vi "Configuration Files.vi"(8 "error in (no error)":errorcluster, 11 "Node Ptr":T3 format="%.0x") -> (0 "error out":errorcluster)   [LabVIEW 2020, in "Ballard ARINC 429 System Explorer.lvlib" / "Implementation.lvlib"]
uses:
  Implementation.lvlib
  <vilib>/NI VeriStand/Custom Device API/Custom Device API.lvlib
  <vilib>/NI VeriStand/Custom Device Tools/Custom Device Utility Library/Custom Device Utility Library.lvlib
  Types/Browse Button.ctl
  Types/Path Control.ctl
  Scripting/Ballard/Ballard ARINC 429 Scripting.lvlib
  <vilib>/NI VeriStand/Custom Device API/Custom Device Item Ref.ctl
  Types/Configuration Files Page Data.ctl
panel:
  in  "Refresh":bool
  in  "Parameters":T1
  in  "Hardware":T1
  in  "SHDocVw.IWebBrowser":refnum<k7>(container)
  in  "General Header":cluster{"Section Name":string}={"Section Name"="Ballard ARINC 429 - Configuration Files"}
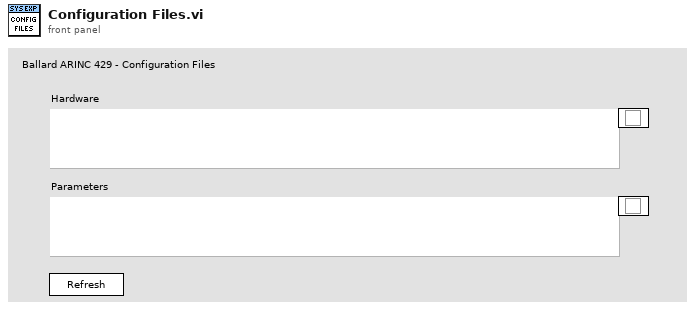
[diagram p1: front panel]
types:
  T1 = typedef "Ballard ARINC 429 System Explorer.lvlib/Implementation.lvlib/Path Control.ctl" = cluster{"file path":path, "Browse":T2}
  T2 = typedef "Ballard ARINC 429 System Explorer.lvlib/Implementation.lvlib/Browse Button.ctl" = bool
  T3 = typedef "Custom Device API.lvlib/Custom Device Item Ref.ctl" = u64
  T4 = typedef "Ballard ARINC 429 System Explorer.lvlib/Implementation.lvlib/Configuration Files Page Data.ctl" = cluster{"Hardware":T1, "Parameters":T1, "most recent parameters path":path, "most recent hardware path":path, "custom device ref":T3, "MD5":string, "CD scripted?":bool, "parameters path ctl ref":refnum<vi>}
  T5 = typedef "Custom Device API.lvlib/Custom Device Commands.ctl" = enum16{"Default", "Item renamed", "Shutdown", "Dynamic button pressed"}
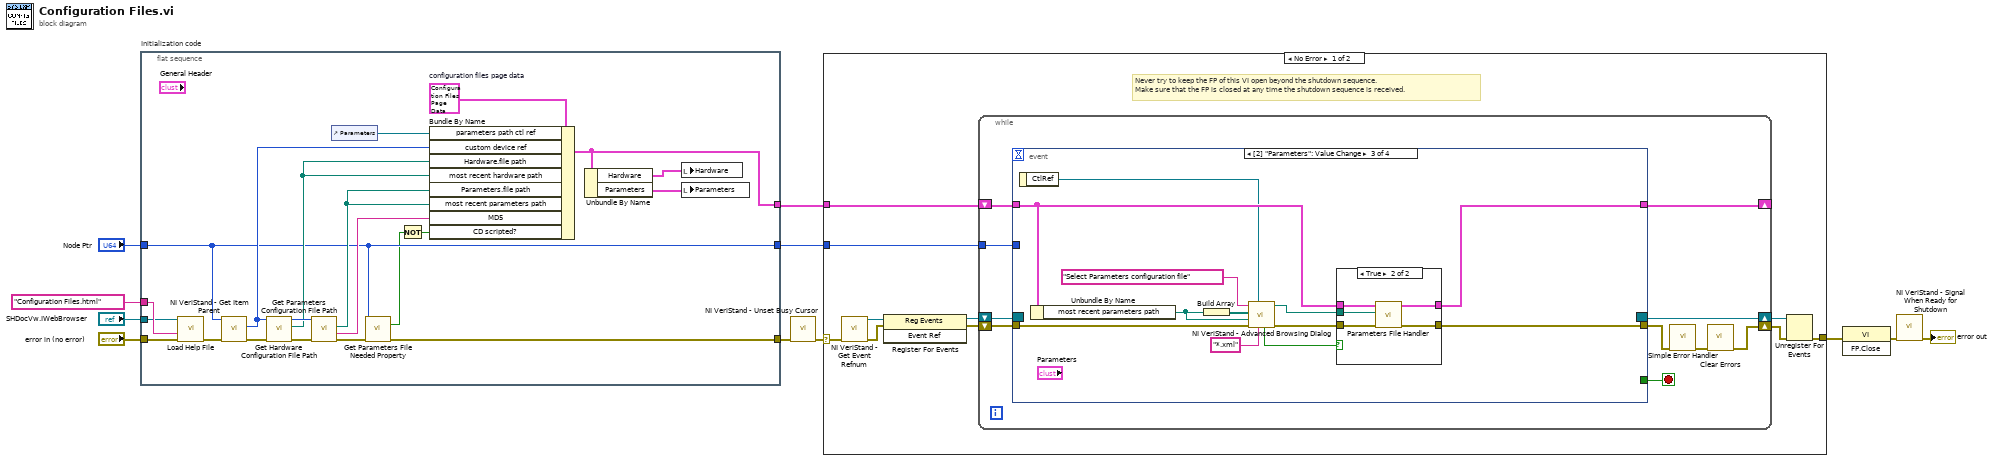
[diagram p0: block diagram]
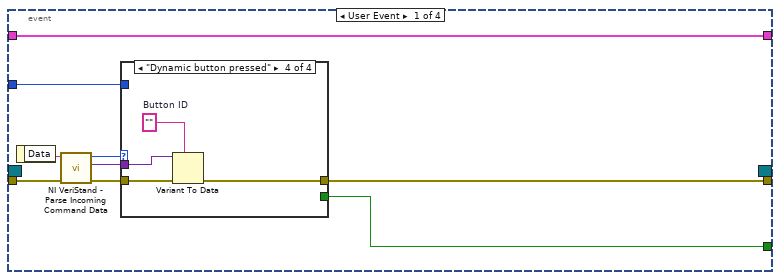
[diagram p2: hidden frame]
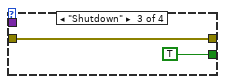
[diagram p5: hidden frame]
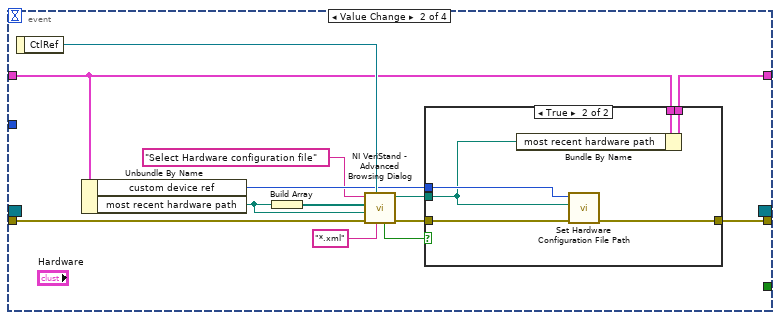
[diagram p6: hidden frame]
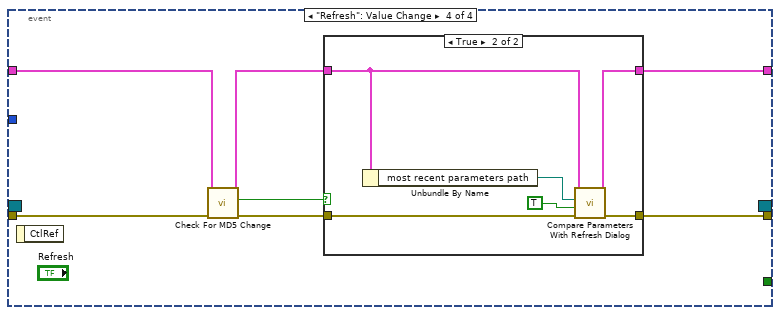
[diagram p9: hidden frame]
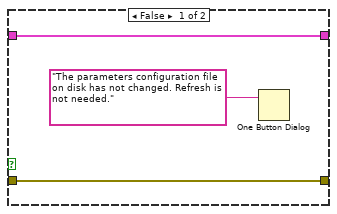
[diagram p10: hidden frame]
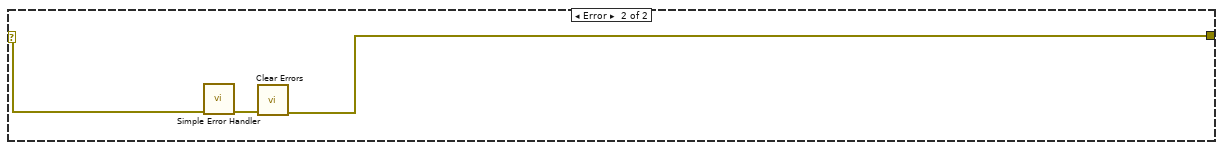
[diagram p11: hidden frame]
diagram:
  n1 = flat-sequence "Initialization code" {
    tunnel: "error in (no error)" -> [w32]
    tunnel: "Node Ptr" -> [w14]
    tunnel: [w15] -> w7
    tunnel: [w14] -> w4
    tunnel: "SHDocVw.IWebBrowser" -> [w21]
    tunnel: "Configuration Files.html" ("CD_CHM_Section") -> [w31]
    tunnel: [w19] -> w1
    frame #0 {
      w30 = T4 {"Hardware"={"file path"=path "", "Browse"=FALSE}, "Parameters"={"file path"=path "", "Browse"=FALSE}, "most recent parameters path"=path "", "most recent hardware path"=path "", "custom device ref"=0, "MD5"="", "CD scripted?"=FALSE, "parameters path ctl ref"=refnum}  # configuration files page data
      n2 = call "Load Help File.vi"("error in (no error)"=w32, "HTML File to Load"=w31, "Browser"=w21) -> ("error out"=w24:errorcluster)  [unwired: 8 in]
      n3 = call <vilib>:"NI VeriStand - Get Item Parent.vi"("error in (no error)"=w24, "Item Ref in"=w14) -> ("error out"=w23:errorcluster, "Parent Ref"=w22:T3)  [unwired: 6 in, 2 out]
      n4 = call "Get Hardware Configuration File Path.vi"("error in"=w23, "Ballard ARINC 429 custom device in"=w22) -> ("error out"=w26:errorcluster, "hardware configuration file path"=w25:path, "Ballard ARINC 429 custom device out"=w27:T3)  [unwired: 6 in, 1 out]
      n5 = call "Get Parameters Configuration File Path.vi"("error in"=w26, "Ballard ARINC 429 custom device in"=w27) -> ("error out"=w16:errorcluster, "MD5 checksum"=w18:string, "parameters configuration file path"=w20:path)  [unwired: 6 in, 1 out]
      n6 = control-ref of="Parameters"() -> (w17:refnum<vi>)
      n7 = call "Get Parameters File Needed Property.vi"("error in"=w16, "configuration files ref"=w14) -> ("error out"=w15:errorcluster, "needed"=w13:bool)  [unwired: 7 in, 1 out]
      n8 = Not(x=w13) -> (.not. x?=w12:bool)
      n9 = Bundle By Name(cluster=w30, "parameters path ctl ref"=w17, "custom device ref"=w22, "Hardware.file path"=w25, "most recent hardware path"=w25, "Parameters.file path"=w20, "most recent parameters path"=w20, "MD5"=w18, "CD scripted?"=w12) -> (w19:T4)
      n10 = Unbundle By Name(w19) -> ("Hardware"=w29:T1, "Parameters"=w28:T1)
      n11 = local write "Hardware"(w29) -> ()
      n12 = local write "Parameters"(w28) -> ()
    }
  }
  n13 = call <vilib>:"NI VeriStand - Unset Busy Cursor.vi"("error in (no error)"=w7) -> ("error out"=w6:errorcluster)  [unwired: 10 out]
  n14 = case shown="No Error" w6 {
    selector: w6 -> [w34 w128]
    tunnel: [w39 w126] -> w11
    tunnel: w4 -> [w35 _]
    tunnel: w1 -> [w33 _]
    frame No Error {
      # "Never try to keep the FP of this VI open beyond the shutdown sequence.\nMake sure that the FP is closed at any time the shutdown sequence is received."
      n15 = call <vilib>:"NI VeriStand - Get Event Refnum.vi"("error in (no error)"=w34) -> ("error out"=w42:errorcluster, "Event Ref"=w38:refnum<user-event>)  [unwired: 9 out]
      n16 = register-events(error in=w42, w38) -> (reference out=w36:refnum<event-registration>, error out=w37:errorcluster)  [unwired: 1 in]
      n17 = while {
        tunnel: w35 -> [w48]
        shift-right: [w45] -> w40
        shift-left: w37 -> [w51]
        shift-right: [w52] -> w41
        shift-left: w36 -> [w50]
        shift-right: [w43] -> _
        shift-left: w33 -> [w44]
        stop <- w49 stop-if-true
        n18 = event shown="[2] \"Parameters\": Value Change" {
          selector: w50 -> [_ _ _ _]
          dyn-events: [_ _ _ _] -> w52
          timeout: _ -> [_ _ _ _]
          tunnel: w51 -> [w61 w82 w102 w113]
          tunnel: [w57 _ _ _] -> w49
          tunnel: [w56 w76 w92 w116] -> w47
          tunnel: w48 -> [w55 _ _ _]
          tunnel: w44 -> [w53 w75 w96 w110]
          tunnel: [w53 w73 w95 w115] -> w43
          event User Event {
            n19 = event-data() -> ("Data"=w60:string)  [unwired: 1 out]
            n20 = call <vilib>:"NI VeriStand - Parse Incoming Command Data.vi"("error in (no error)"=w61, "Incoming data"=w60) -> ("error out"=w59:errorcluster, "Outgoing data"=w54:variant, "Action"=w58:T5)  [unwired: 7 out]
            n21 = case shown="\"Dynamic button pressed\"" w58 {
              tunnel: w59 -> [w62 w63 w64 w69]
              tunnel: [_ _ TRUE _] -> w57
              tunnel: [w62 w63 w64 w66] -> w56
              tunnel: w55 -> [_ _ _ _]
              tunnel: w54 -> [_ _ _ w68]
              frame "Default", Default {
              }
              frame "Item renamed" {
              }
              frame "Shutdown" {
              }
              frame "Dynamic button pressed" {
                w67 = ""  # Button ID
                n22 = Variant To Data(error in=w69, type=w67, Variant=w68) -> (error out=w66:errorcluster)  [unwired: 1 out]
              }
            }
          }
          event Value Change {
            n23 = event-data() -> ("CtlRef"=w80:refnum<vi>)  [unwired: 1 out]
            n24 = Unbundle By Name(w75) -> ("custom device ref"=w71:T3, "most recent hardware path"=w78:path)
            n25 = Build Array(w78) -> (w79:path[])
            n26 = call <vilib>:"NI VeriStand - Advanced Browsing Dialog.vi"("File Pattern"="*.xml", "CtlRef"=w80, "error in (no error)"=w82, "Most recent path"=w78, "Paths"=w79, "Dialog Title"="Select Hardware configuration file") -> ("error out"=w77:errorcluster, "Selected file"=w74:path, "Valid?"=w72:bool)  [unwired: 2 in, 1 out]
            n27 = case shown="True" w72 {
              tunnel: w77 -> [w84 w90]
              tunnel: w71 -> [_ w89]
              tunnel: [w84 w88] -> w76
              tunnel: w75 -> [w83 w87]
              tunnel: w74 -> [_ w86]
              tunnel: [w83 w85] -> w73
              frame False {
              }
              frame True {
                n28 = Bundle By Name(cluster=w87, "most recent hardware path"=w86) -> (w85:T4)
                n29 = call "Set Hardware Configuration File Path.vi"("error in"=w90, "hardware configuration file path"=w86, "Ballard ARINC 429 custom device in"=w89) -> ("error out"=w88:errorcluster)  [unwired: 7 in, 1 out]
              }
            }
          }
          event Value Change {
            n30 = event-data() -> ("CtlRef"=w94:refnum<vi>)  [unwired: 1 out]
            n31 = Unbundle By Name(w96) -> ("most recent parameters path"=w98:path)
            n32 = Build Array(w98) -> (w100:path[])
            n33 = call <vilib>:"NI VeriStand - Advanced Browsing Dialog.vi"("File Pattern"="*.xml", "CtlRef"=w94, "error in (no error)"=w102, "Most recent path"=w98, "Paths"=w100, "Dialog Title"="Select Parameters configuration file") -> ("error out"=w97:errorcluster, "Selected file"=w93:path, "Valid?"=w91:bool)  [unwired: 2 in, 1 out]
            n34 = case shown="True" w91 {
              tunnel: w97 -> [w103 w109]
              tunnel: w96 -> [w104 w108]
              tunnel: [w104 w107] -> w95
              tunnel: w93 -> [_ w106]
              tunnel: [w103 w105] -> w92
              frame False {
              }
              frame True {
                n35 = call "Parameters File Handler.vi"("error in"=w109, "selected parameters file"=w106, "configuration files page data"=w108) -> ("error out"=w105:errorcluster, "configuration files page data out"=w107:T4)  [unwired: 7 in]
              }
            }
          }
          event "Refresh": Value Change {
            n36 = event-data() -> ()  [unwired: 2 out]
            n37 = call "Check For MD5 Change.vi"("error in"=w113, "configuration files page data"=w110) -> ("error out"=w112:errorcluster, "MD5 change?"=w111:bool, "configuration files page data out"=w114:T4)  [unwired: 7 in]
            n38 = case shown="True" w111 {
              tunnel: [w118 w125] -> w116
              tunnel: w112 -> [w118 w124]
              tunnel: w114 -> [w117 w123]
              tunnel: [w117 w121] -> w115
              frame False {
                n39 = One Button Dialog(message="The parameters configuration file on disk has not changed. Refresh is not needed.") -> ()  [unwired: 1 in, 1 out]
              }
              frame True {
                n40 = Unbundle By Name(w123) -> ("most recent parameters path"=w122:path)
                n41 = call "Compare Parameters With Refresh Dialog.vi"("error in"=w124, "refresh button"=TRUE, "selected parameters file"=w122, "configuration files page data"=w123) -> ("error out"=w125:errorcluster, "configuration files page data out"=w121:T4)  [unwired: 6 in]
              }
            }
          }
        }
        n42 = call <vilib>:"Simple Error Handler.vi"("error in (no error)"=w47) -> ("error out"=w46:errorcluster)  [unwired: 1 in, 7 out]
        n43 = call <vilib>:"Clear Errors.vi"("error in (no error)"=w46) -> ("error out"=w45:errorcluster)  [unwired: 1 in, 5 out]
      }
      n44 = Unregister For Events(event registration refnum=w41, error in=w40) -> (error out=w39:errorcluster)
    }
    frame Error {
      n45 = call <vilib>:"Simple Error Handler.vi"("error in (no error)"=w128) -> ("error out"=w127:errorcluster)  [unwired: 1 in, 7 out]
      n46 = call <vilib>:"Clear Errors.vi"("error in (no error)"=w127) -> ("error out"=w126:errorcluster)  [unwired: 1 in, 5 out]
    }
  }
  n47 = invoke class="VI" method="FP.Close"(error in=w11) -> (error out=w10:errorcluster)  [unwired: 2 in, 2 out]
  n48 = call <vilib>:"NI VeriStand - Signal When Ready for Shutdown.vi"("error in (no error)"=w10) -> ("error out"=→"error out":errorcluster)  [unwired: 10 out]
